vi "Abort Sequence.vi"(8 "error in":errorcluster, 10 "reason":string, 11 "Sequence Executor in":refnum<class "Sequence Executor.lvclass">) -> (0 "error out":errorcluster, 3 "Sequence Executor out":refnum<class "Sequence Executor.lvclass">)   [LabVIEW 2026, in "Sequence Executor.lvclass"]
doc: "PRIVATE. Marks Results[Step Index] ABORTED with the given reason, applies safe setpoints to the rig, Running F, Overall Verdict ABORTED, Status ABORTED: reason, refreshes displays. No-op when not running."
uses:
  Sequence Executor.lvclass
  Sequence Executor.lvclass/Sequence Executor.ctl
  Rig Messages/Apply Setpoints Msg/Apply Setpoints Msg.lvclass/Apply Setpoints Msg.ctl
  <vilib>/ActorFramework/Message Enqueuer/Message Enqueuer.lvclass/Message Enqueuer.ctl
  <vilib>/ActorFramework/Message Enqueuer/Enqueue.vi
  Rig Messages/Apply Setpoints Msg/Apply Setpoints Msg.lvclass
  <vilib>/ActorFramework/Message Priority Queue/Priority Enqueue.vi
  <vilib>/ActorFramework/Message Enqueuer/Message Enqueuer.lvclass
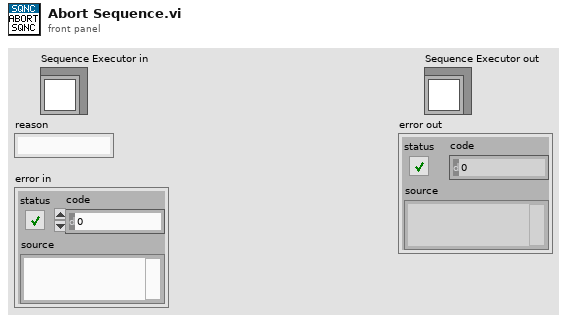
[diagram p1: front panel]
types:
  T1 = typedef "Step Result.ctl" = cluster{"step_no":i32, "step_name":string, "result":string, "reason":string, "measured":dbl, "target":dbl, "duration_ms":dbl}
  T2 = typedef "Rig Config.ctl" = cluster{"rig_id":string, "description":string, "plugin_class":string, "channels":T3[]}
  T3 = typedef "Channel Definition.ctl" = cluster{"name":string, "unit":string, "min":dbl, "max":dbl}
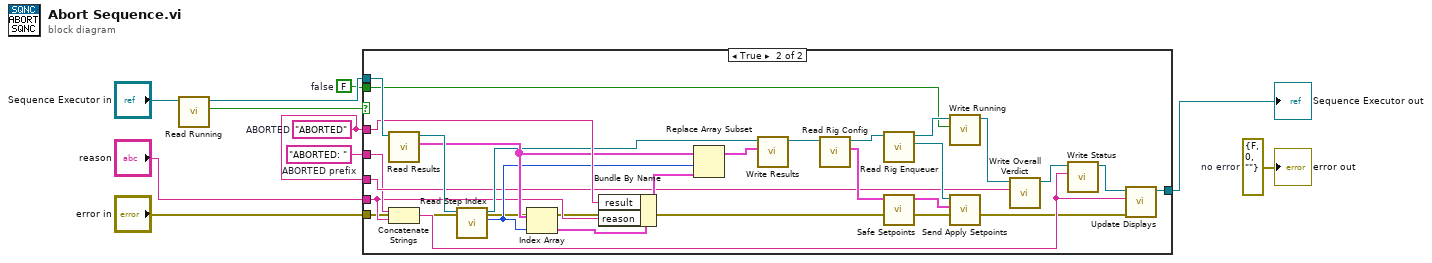
[diagram p0: block diagram]
diagram:
  w5 = "ABORTED: "  # ABORTED prefix
  w6 = "ABORTED"  # ABORTED
  w7 = FALSE  # false
  w1 = errorcluster {"status"=FALSE, "code"=0, "source"=""}  # no error
  n1 = call "Read Running.vi"("Sequence Executor in"="Sequence Executor in") -> ("Running"=w3:bool, "Sequence Executor out"=w9:refnum<class "Sequence Executor.lvclass">)  [unwired: 8 in, 1 out]
  n2 = case shown="True" w3 {
    tunnel: w9 -> [w11 w36]
    tunnel: "reason" -> [_ w17]
    tunnel: [w11 w12] -> w2
    tunnel: w6 -> [_ w34]
    tunnel: w7 -> [_ w21]
    tunnel: w6 -> [_ w19]
    tunnel: w5 -> [_ w18]
    tunnel: "error in" -> [_ w13]
    frame False {
    }
    frame True {
      n3 = call "Read Results.vi"("Sequence Executor in"=w36) -> ("Results"=w32:T1[], "Sequence Executor out"=w35:refnum<class "Sequence Executor.lvclass">)  [unwired: 8 in, 1 out]
      n4 = Concatenate Strings(w18, w17) -> (w14:string)
      n5 = call "Read Step Index.vi"("Sequence Executor in"=w35) -> ("Step Index"=w31:i32, "Sequence Executor out"=w29:refnum<class "Sequence Executor.lvclass">)  [unwired: 8 in, 1 out]
      n6 = Index Array(array=w32, index=w31) -> (element=w33:T1)
      n7 = Bundle By Name(cluster=w33, "result"=w34, "reason"=w17) -> (w30:T1)
      n8 = Replace Array Subset(array=w32, new element=w30, index=w31) -> (w28:T1[])
      n9 = call "Write Results.vi"("Results"=w28, "Sequence Executor in"=w29) -> ("Sequence Executor out"=w27:refnum<class "Sequence Executor.lvclass">)  [unwired: 8 in, 1 out]
      n10 = call "Read Rig Config.vi"("Sequence Executor in"=w27) -> ("Rig Config"=w26:T2, "Sequence Executor out"=w25:refnum<class "Sequence Executor.lvclass">)  [unwired: 8 in, 1 out]
      n11 = call "Read Rig Enqueuer.vi"("Sequence Executor in"=w25) -> ("Actor Framework:Message Enqueuer"=w24:refnum<class "Message Enqueuer.lvclass">, "Sequence Executor out"=w22:refnum<class "Sequence Executor.lvclass">)  [unwired: 8 in, 1 out]
      n12 = call "Safe Setpoints.vi"("Rig Config"=w26) -> ("setpoints"=w23:cluster{"channel":string, "value":dbl}[])  [unwired: 10 in]
      n13 = call "Write Running.vi"("Running"=w21, "Sequence Executor in"=w22) -> ("Sequence Executor out"=w20:refnum<class "Sequence Executor.lvclass">)  [unwired: 8 in, 1 out]
      n14 = call "Send Apply Setpoints.vi"("setpoints"=w23, "Message Enqueuer"=w24) -> ()  [unwired: 8 in, 2 out]
      n15 = call "Write Overall Verdict.vi"("Overall Verdict"=w19, "Sequence Executor in"=w20) -> ("Sequence Executor out"=w16:refnum<class "Sequence Executor.lvclass">)  [unwired: 8 in, 1 out]
      n16 = call "Write Status.vi"("Status"=w14, "Sequence Executor in"=w16) -> ("Sequence Executor out"=w15:refnum<class "Sequence Executor.lvclass">)  [unwired: 8 in, 1 out]
      n17 = call "Update Displays.vi"("error in"=w13, "Status"=w14, "Sequence Executor in"=w15) -> ("Sequence Executor out"=w12:refnum<class "Sequence Executor.lvclass">)  [unwired: 7 in, 1 out]
    }
  }
  "Sequence Executor out" <- w2
  "error out" <- w1
